vi "控件文本.vi"(6 "数组":string[][](array[string]), 9 "字号":u32, 10 "选择列":i32, 11 "引用":refnum<vi>) -> ()   [LabVIEW 2025]
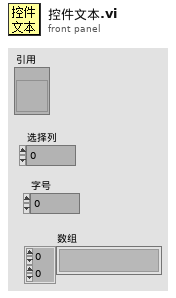
[diagram p1: front panel]
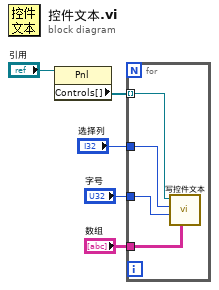
[diagram p0: block diagram]
diagram:
  n1 = property class="Pnl"(reference="引用") -> ("Controls[]"=w1:refnum<vi>[])  [unwired: 1 in, 2 out]
  n2 = for {
    tunnel: w1 -> [w9] mode=indexing
    tunnel: "数组" -> [w6]
    tunnel: "选择列" -> [w8]
    tunnel: "字号" -> [w7]
    n3 = call "写控件文本.vi"("数组"=w6, "字号"=w7, "选择列"=w8, "引用"=w9) -> ()  [unwired: 8 in]
  }
